vi "zs_prologer.vi"(5 "goal_y":dbl=300.0, 6 "goal_x":dbl=520.0, 7 "goal_node":string="c400", 8 "y":dbl=3.6, 9 "x":dbl=51.0) -> (3 "goal_array":T1(array[cluster]))   [LabVIEW 2014, in "Dialogue.lvlib" / "Dialogue.lvclass"]
uses:
  Dialogue.lvclass
  Global_var/Global_var.vi
panel:
  out "字符串":string
  out "坐标数组":dbl[][](array[numeric])
  out "添加的路径":path
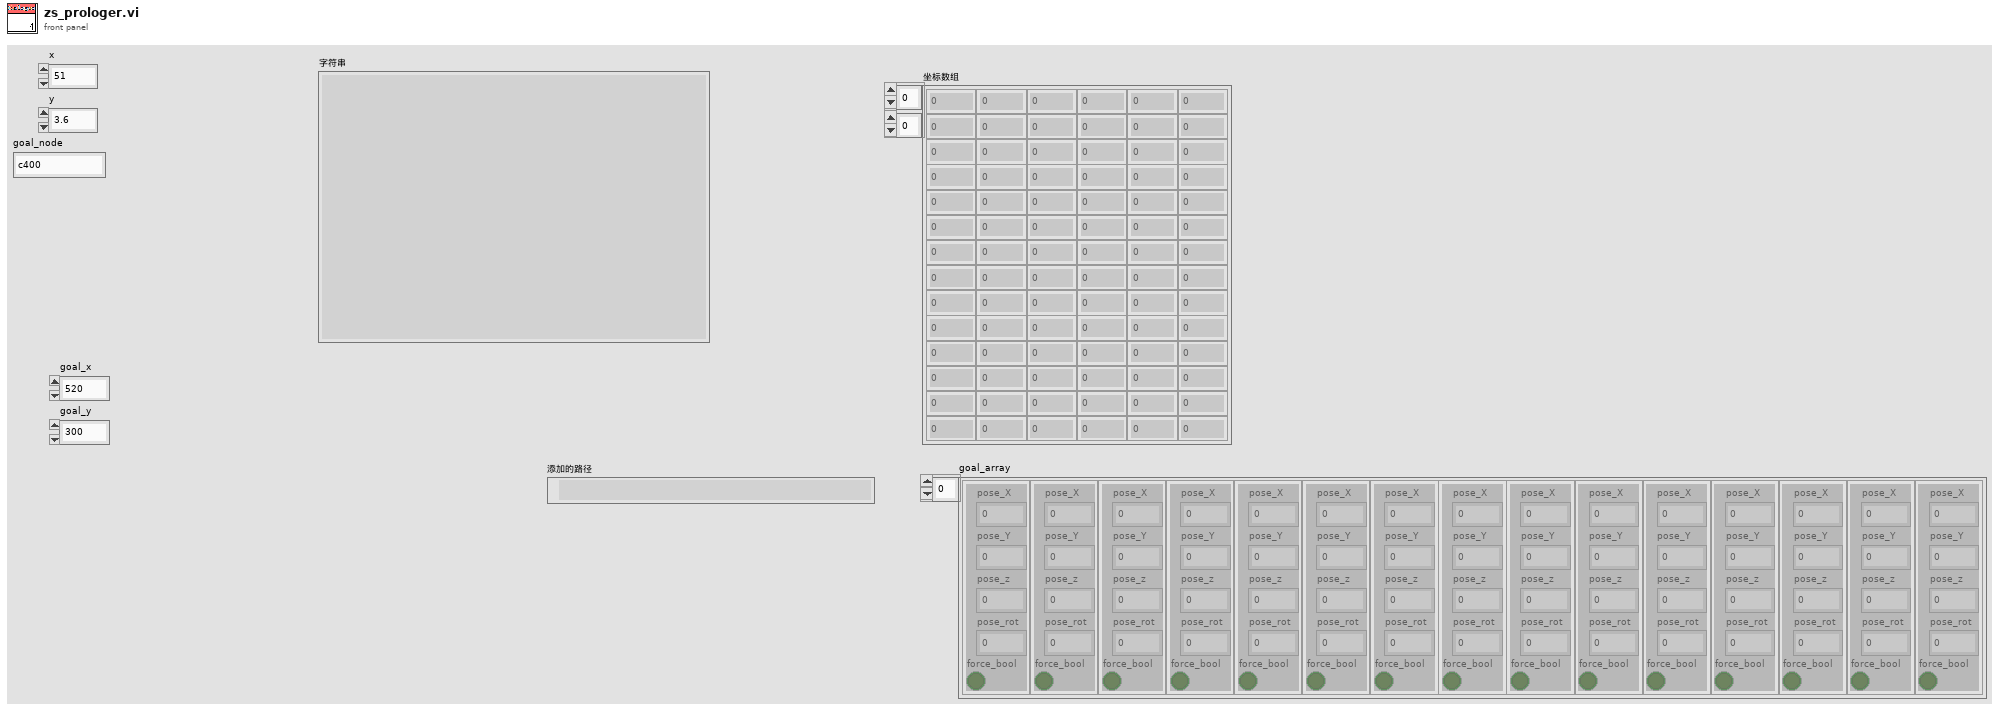
[diagram p1: front panel]
types:
  T1 = cluster{"pose_X":dbl, "pose_Y":dbl, "pose_z":dbl, "pose_rot":dbl, "force_bool":bool}[]
  T2 = cluster{"pose_X":dbl, "pose_Y":dbl, "pose_z":dbl, "pose_rot":dbl, "force_bool":bool}
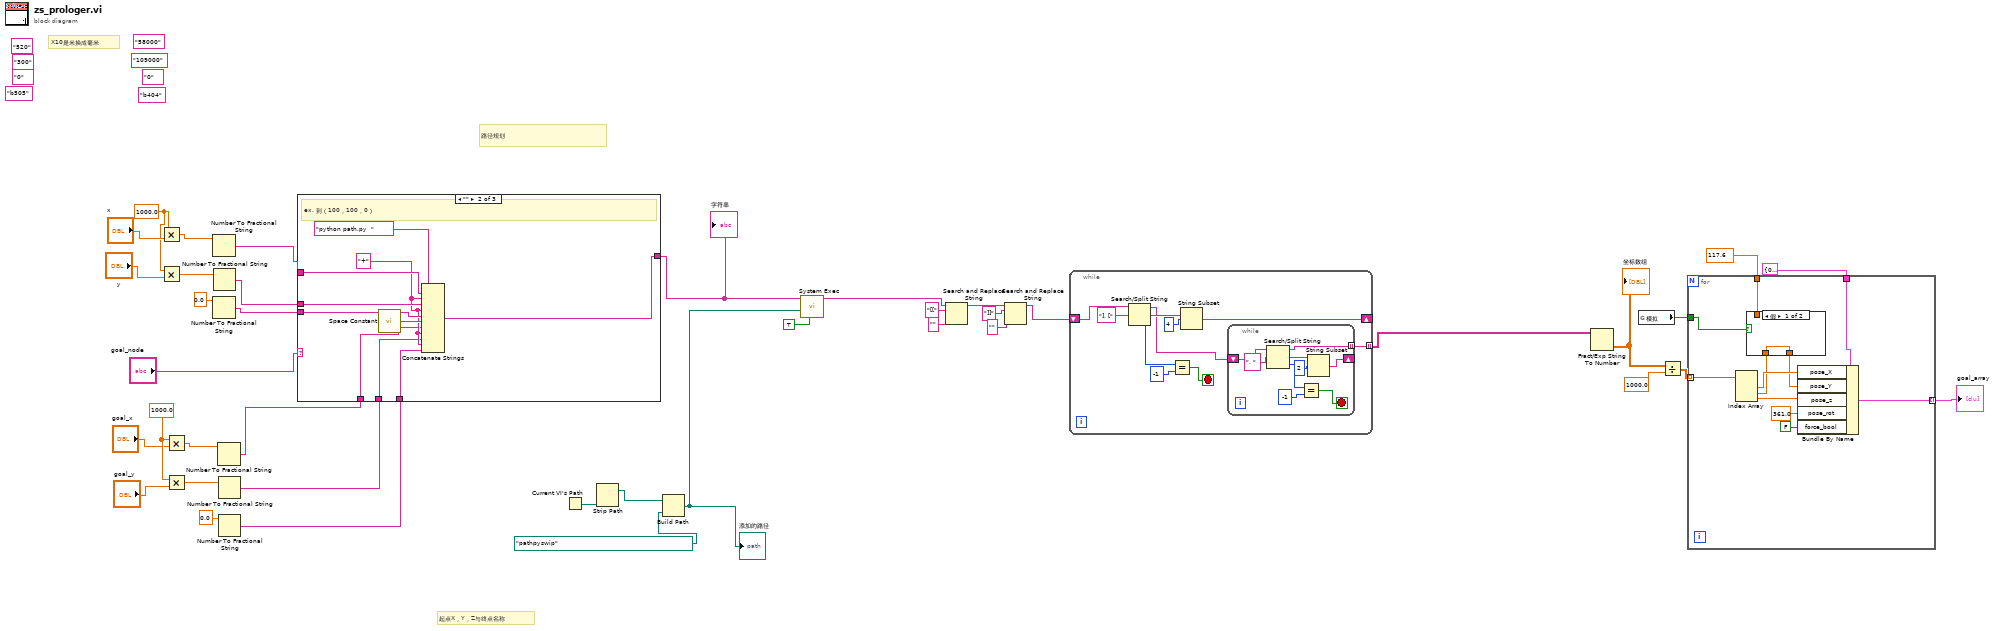
[diagram p0: block diagram]
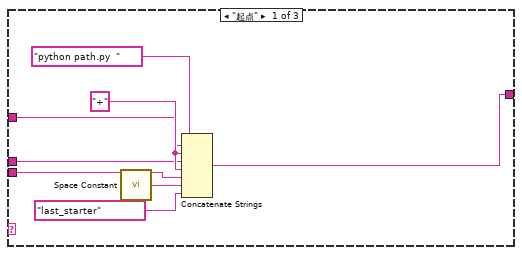
[diagram p2: hidden frame]
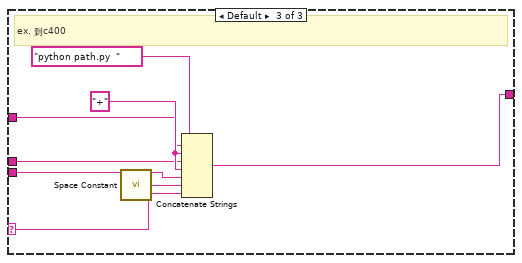
[diagram p3: hidden frame]
diagram:
  w11 = 1000.0 ("x")
  (unwired) "0" ("元素")
  (unwired) "b404" ("元素")
  (unwired) "109000" ("元素")
  (unwired) "58000" ("元素")
  w30 = 1000.0 ("x")
  (unwired) "b505" ("元素")
  (unwired) "0" ("元素")
  (unwired) "300" ("元素")
  (unwired) "520" ("元素")
  # "X10是米换成毫米"
  # "起点X，Y，Z与终点名称"
  # "路径规划"
  n1 = Multiply(x=w30, y="x") -> (x*y=w29:dbl)
  n2 = Multiply(x=w30, y="y") -> (x*y=w28:dbl)
  n3 = Multiply(x=w11, y="goal_x") -> (x*y=w12:dbl)
  n4 = Multiply(x=w11, y="goal_y") -> (x*y=w13:dbl)
  n5 = Number To Fractional String(number=w29) -> (F-format string=w7:string)  [unwired: 3 in]
  n6 = Number To Fractional String(number=0.0 ("数字")) -> (F-format string=w5:string)  [unwired: 3 in]
  n7 = Number To Fractional String(number=w28) -> (F-format string=w6:string)  [unwired: 3 in]
  n8 = Number To Fractional String(number=w12) -> (F-format string=w3:string)  [unwired: 3 in]
  n9 = Number To Fractional String(number=w13) -> (F-format string=w2:string)  [unwired: 3 in]
  n10 = Number To Fractional String(number=0.0 ("数字")) -> (F-format string=w1:string)  [unwired: 3 in]
  n11 = case shown="\"\"" "goal_node" {
    selector: "goal_node" -> [_ _ w59]
    tunnel: [w41 w53 w60] -> w4
    tunnel: w7 -> [w45 w56 w63]
    tunnel: w6 -> [w44 w55 w62]
    tunnel: w5 -> [w43 w54 w61]
    tunnel: w3 -> [_ w51 _]
    tunnel: w2 -> [_ w50 _]
    tunnel: w1 -> [_ w49 _]
    frame "起点" {
      w47 = "+"
      n12 = call <vilib>:"Space Constant.vi"() -> ("String"=w46:string)
      n13 = Concatenate Strings("python path.py  " ("command line"), w45, w47, w44, w47, w43, w46, "last_starter" ("command line")) -> (w41:string)
    }
    frame "" {
      w52 = "+"
      # "ex. 到（100，100，0）"
      n14 = call <vilib>:"Space Constant.vi"() -> ("String"=w57:string)
      n15 = Concatenate Strings("python path.py  " ("command line"), w56, w52, w55, w52, w54, w57, w51, w52, w50, w52, w49) -> (w53:string)
    }
    frame Default {
      w65 = "+"
      # "ex. 到c400"
      n16 = call <vilib>:"Space Constant.vi"() -> ("String"=w64:string)
      n17 = Concatenate Strings("python path.py  " ("command line"), w63, w65, w62, w65, w61, w64, w59) -> (w60:string)
    }
  }
  "字符串" <- w4
  n18 = Current VI's Path() -> (path=w40:path)
  n19 = Strip Path(path=w40) -> (stripped path=w38:path)  [unwired: 1 out]
  n20 = Build Path(base path=w38, name or relative path=path "pathpyswip") -> (appended path=w36:path)
  "添加的路径" <- w36
  n21 = call <vilib>:"System Exec.vi"("run minimized? (F)"=TRUE, "working directory"=w36, "command line"=w4) -> ("standard output"=w17:string)  [unwired: 5 in, 3 out]
  n22 = Search and Replace String(input string=w17, search string="[[" ("搜索字符串"), replace string="" ("替换字符串(\"\")")) -> (result string=w22:string)  [unwired: 5 in, 3 out]
  n23 = Search and Replace String(input string=w22, search string="]]" ("搜索字符串"), replace string="" ("替换字符串(\"\")")) -> (result string=w20:string)  [unwired: 5 in, 3 out]
  n24 = while {
    shift-right: [w72] -> _
    shift-left: w20 -> [w76]
    tunnel: [w68] -> w16 mode=indexing
    stop <- w67 stop-if-true
    n25 = Search/Split String(string=w76, search string/char (-)="], [" ("搜索字符串")) -> (substring before match=w69:string, match + rest of string=w74:string, offset of match=w71:i32)  [unwired: 1 in]
    n26 = Equal?(x=w71, y=-1) -> (x = y?=w67:bool)
    n27 = String Subset(string=w74, offset (0)=4 ("偏移量(0)")) -> (substring=w72:string)  [unwired: 1 in]
    n28 = while {
      shift-right: [w82] -> _
      shift-left: w69 -> [w85]
      tunnel: [w80] -> w68 mode=indexing
      stop <- w77 stop-if-true
      n29 = Search/Split String(string=w85, search string/char (-)=", " ("搜索字符串/字符(-)")) -> (substring before match=w80:string, match + rest of string=w81:string, offset of match=w78:i32)  [unwired: 1 in]
      n30 = Equal?(x=w78, y=-1) -> (x = y?=w77:bool)
      n31 = String Subset(string=w81, offset (0)=2 ("偏移量(0)")) -> (substring=w82:string)  [unwired: 1 in]
    }
  }
  n32 = Fract/Exp String To Number(string=w16) -> (number=w26:dbl[][])  [unwired: 3 in, 1 out]
  "坐标数组" <- w26
  n33 = global read "Global_var.vi" "模拟"() -> (w15:bool)
  n34 = Divide(x=w26, y=1000.0) -> (x/y=w27:dbl[][])
  n35 = for {
    tunnel: T2 {"pose_X"=0.0, "pose_Y"=0.0, "pose_z"=0.0, "pose_rot"=0.0, "force_bool"=FALSE} ("goal_with_force") -> [w93]
    tunnel: [w91] -> w33 mode=indexing
    tunnel: w27 -> [w90] mode=indexing
    tunnel: w15 -> [w88]
    tunnel: 117.6 ("x") -> [w86]
    n36 = Index Array(array=w90) -> (element #1=w96:dbl, element #2=w89:dbl, element #3=w95:dbl)  [unwired: 3 in]
    n37 = case shown="假" w88 {
      tunnel: w89 -> [w97 w98]
      tunnel: [w97 w98] -> w87
      tunnel: w86 -> [_ _]
      frame False {
      }
      frame True {
      }
    }
    n38 = Bundle By Name(cluster=w93, "pose_X"=w96, "pose_Y"=w87, "pose_z"=w95, "pose_rot"=361.0, "force_bool"=FALSE) -> (w91:T2)
  }
  "goal_array" <- w33
